vi "Initialize instruments.vi"(0 "HIPOT":refnum<visa-resource-name>="COM62", 1 "Barcode":refnum<visa-resource-name>) -> (6 "Power supply":errorcluster, 7 "error out":errorcluster)   [LabVIEW 2021]
uses:
  Main_VI/HI-POT_Driver/Hi-pot_Driver.ctl
  Main_VI/Control/Barcode.ctl
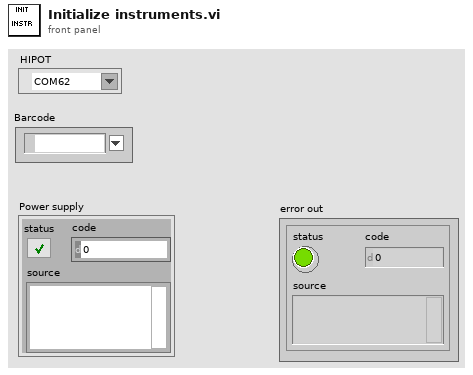
[diagram p1: front panel]
types:
  T1 = typedef "Barcode.ctl" = enum16{"Init", "Read", "Stop Reading", "Clear", "Close"}
  T2 = typedef "Hi-pot_Driver.ctl" = enum16{"Init ", "Interlock status", "Set UP DCW", "Set UP ACW", "Set UP IR", "Read", "Clear", "Close"}
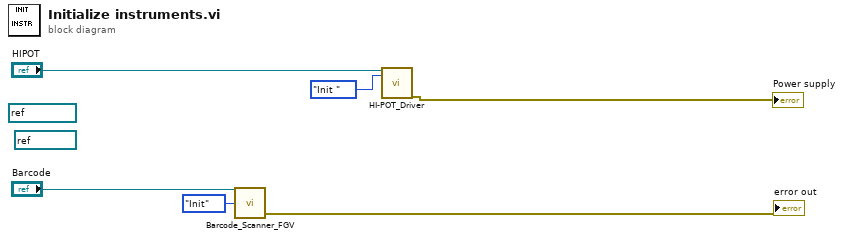
[diagram p0: block diagram]
diagram:
  (unwired) refnum<visa-resource-name> "COM7" ("COM")
  (unwired) refnum<visa-resource-name> "COM15" ("VISA resource name")
  n1 = call "Barcode_Scanner_FGV.vi"("Action"=Barcode."Init", "COM"="Barcode") -> ("error out"=→"error out":errorcluster)  [unwired: 1 in, 2 out]
  n2 = call "HI-POT_Driver.vi"("VISA resource name"="HIPOT", 1:Hi-pot_Driver."Init ") -> ("error out"=→"Power supply":errorcluster)  [unwired: 7 in, 10 out]
